vi "Parse Call Handover Param.vi"(8 "error in (no error)":errorcluster caption="에러 입력(에러 없음)", 10 "JSON string":string, 11 "Instrument Manager 입력":refnum<class "Instrument Manager.lvclass">) -> (0 "error out":errorcluster caption="에러 출력", 1 "NR Call Handover Param":T2, 2 "Call Handover Param":T1, 3 "Instrument Manager 출력":refnum<class "Instrument Manager.lvclass">)   [LabVIEW 2023, in "Instrument Manager.lvclass"]
uses:
  Instrument Manager.lvclass
  Type Definition/NR Call Handover Param.ctl
  Module/ANRITSU Call Box/Type Definition/NR Modulation Type.ctl
  Call Handover Param.ctl
  Instrument Manager.lvclass/Instrument Manager.ctl
  Module/ANRITSU Call Box/ANRITSU Call Box.lvlib
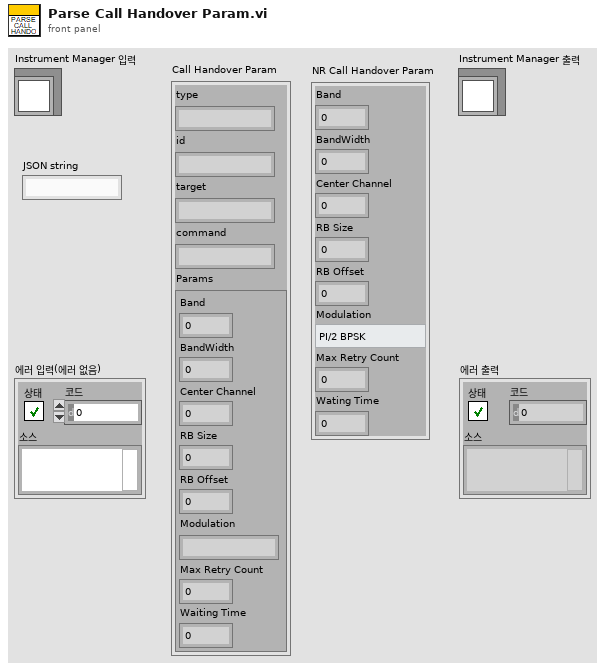
[diagram p1: front panel]
types:
  T1 = typedef "Instrument Manager.lvclass/Call Handover Param.ctl" = cluster{"type":string, "id":string, "target":string, "command":string, "Params":cluster{"Band":u32, "BandWidth":u32, "Center Channel":u32, "RB Size":i32, "RB Offset":i32, "Modulation":string, "Max Retry Count":i32, "Waiting Time":i32}}
  T2 = typedef "NR Call Handover Param.ctl" = cluster{"Band":u32, "BandWidth":u32, "Center Channel":u32, "RB Size":i32, "RB Offset":i32, "Modulation":T3, "Max Retry Count":i32, "Wating Time":i32}
  T3 = typedef "ANRITSU Call Box.lvlib/NR Modulation Type.ctl" = enum16{"PI/2 BPSK", "QPSK", "16QAM", "64QAM", "256QAM"}
  T4 = cluster{"Band":u32, "BandWidth":u32, "Center Channel":u32, "RB Size":i32, "RB Offset":i32, "Modulation":string, "Max Retry Count":i32, "Waiting Time":i32}
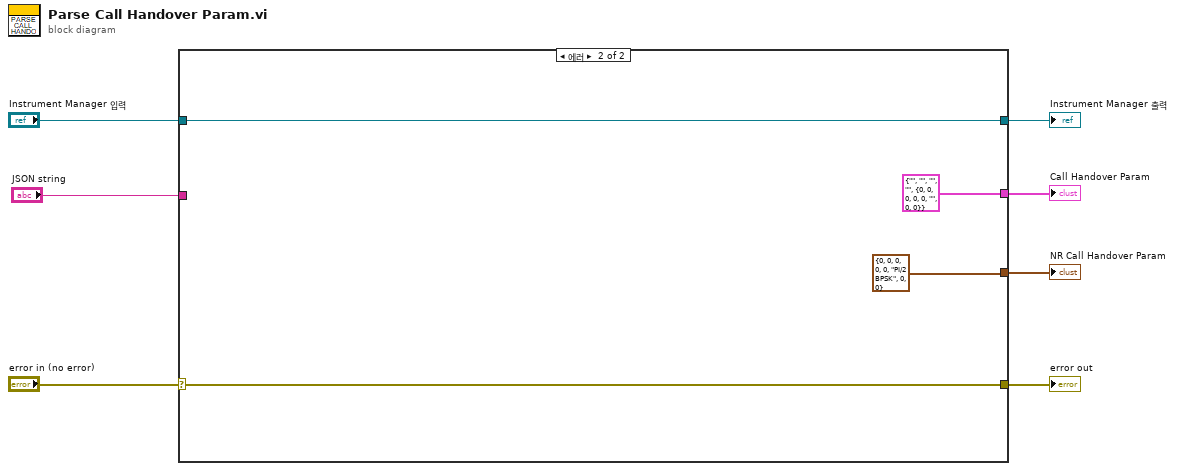
[diagram p0: block diagram]
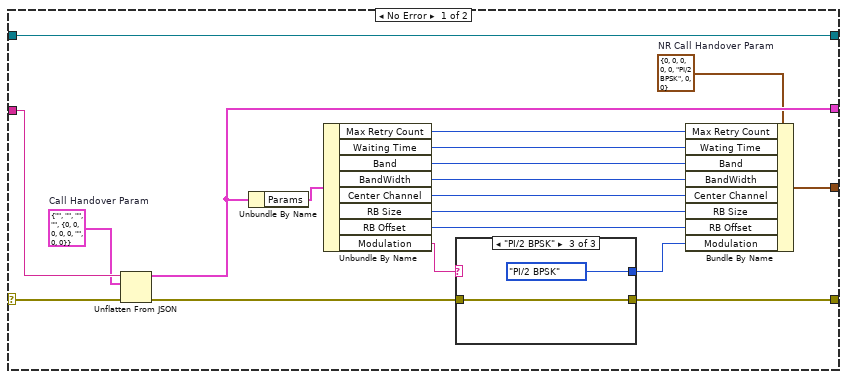
[diagram p2: hidden frame]
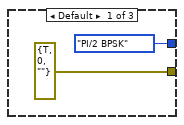
[diagram p3: hidden frame]
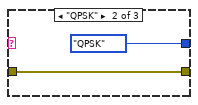
[diagram p4: hidden frame]
diagram:
  n1 = case shown="에러" "error in (no error)" {
    selector: "error in (no error)" -> [w24 w36]
    tunnel: [w13 w36] -> w3
    tunnel: [w26 w35] -> w4
    tunnel: "Instrument Manager 입력" -> [w26 w35]
    tunnel: "JSON string" -> [w25 _]
    tunnel: [w10 T1 {"type"="", "id"="", "target"="", "command"="", "Params"={"Band"=0, "BandWidth"=0, "Center Channel"=0, "RB Size"=0, "RB Offset"=0, "Modulation"="", "Max Retry Count"=0, "Waiting Time"=0}} ("Call Handover Param")] -> w1
    tunnel: [w8 T2 {"Band"=0, "BandWidth"=0, "Center Channel"=0, "RB Size"=0, "RB Offset"=0, "Modulation"=enum."PI/2 BPSK", "Max Retry Count"=0, "Wating Time"=0} ("NR Call Handover Param")] -> w2
    frame No Error {
      w9 = T2 {"Band"=0, "BandWidth"=0, "Center Channel"=0, "RB Size"=0, "RB Offset"=0, "Modulation"=enum."PI/2 BPSK", "Max Retry Count"=0, "Wating Time"=0}  # NR Call Handover Param
      w11 = T1 {"type"="", "id"="", "target"="", "command"="", "Params"={"Band"=0, "BandWidth"=0, "Center Channel"=0, "RB Size"=0, "RB Offset"=0, "Modulation"="", "Max Retry Count"=0, "Waiting Time"=0}}  # Call Handover Param
      n2 = Unflatten From JSON(JSON string=w25, type and defaults=w11, error in (no error)=w24) -> (value=w10:T1, error out=w15:errorcluster)  [unwired: 4 in]
      n3 = Unbundle By Name(w10) -> ("Params"=w23:T4)
      n4 = Unbundle By Name(w23) -> ("Max Retry Count"=w12:i32, "Waiting Time"=w21:i32, "Band"=w20:u32, "BandWidth"=w19:u32, "Center Channel"=w18:u32, "RB Size"=w17:i32, "RB Offset"=w16:i32, "Modulation"=w22:string)
      n5 = case shown="\"PI/2 BPSK\"" w22 {
        tunnel: w15 -> [_ w29 w31]
        tunnel: [NR_Modulation_Type."PI/2 BPSK" ("Modulation") NR_Modulation_Type."QPSK" ("Modulation") NR_Modulation_Type."PI/2 BPSK" ("Modulation")] -> w14
        tunnel: [errorcluster {"status"=TRUE, "code"=0, "source"=""} ("error out") w29 w31] -> w13
        frame Default {
        }
        frame "QPSK" {
        }
        frame "PI/2 BPSK" {
        }
      }
      n6 = Bundle By Name(cluster=w9, "Max Retry Count"=w12, "Wating Time"=w21, "Band"=w20, "BandWidth"=w19, "Center Channel"=w18, "RB Size"=w17, "RB Offset"=w16, "Modulation"=w14) -> (w8:T2)
    }
    frame Error {
    }
  }
  "error out" <- w3
  "Instrument Manager 출력" <- w4
  "Call Handover Param" <- w1
  "NR Call Handover Param" <- w2
